vi "VIH HelpGen - Build - Project File Paths Container.vi"(6 "cmd (get)":enum16{"get", "set"}(ring), 9 "HTML Paths in":path[](array[path]), 11 "Item Paths in":path[](array[path])) -> (1 "HTML Paths":path[](array[path]), 2 "Item File Names":string[](array[string]), 3 "Item Paths":path[](array[path]))   [LabVIEW 2014]
doc: "::: VI Helpeks :::\nCopyright (c) 2000-2026 Konstantin Shifershteyn. All rights reserved."
panel:
  # "VI Helpeks\nCopyright (c) 2012-2026 Konstantin Shifershteyn"
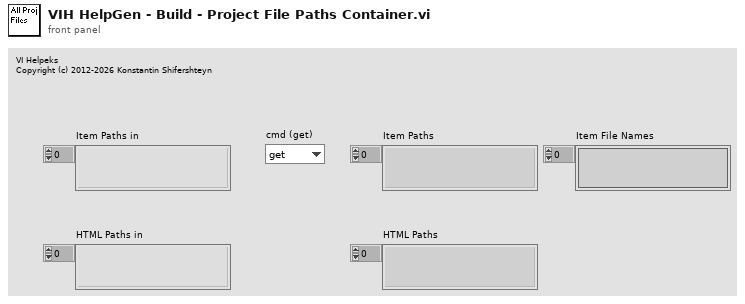
[diagram p1: front panel]
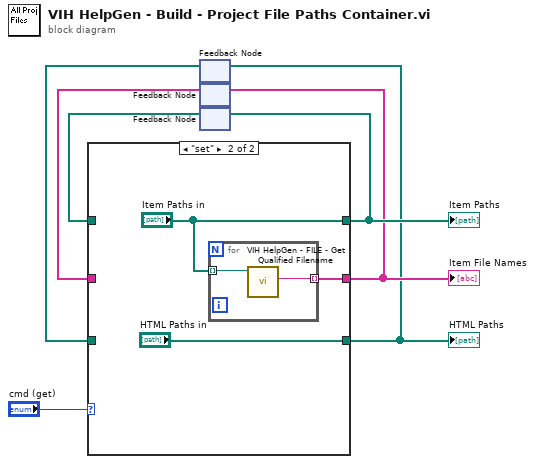
[diagram p0: block diagram]
diagram:
  n1 = feedback #1() -> (w1:path[])  [unwired: 1 in]
  n2 = feedback #2() -> (w3:string[])  [unwired: 1 in]
  n3 = feedback #3() -> (w5:path[])  [unwired: 1 in]
  n4 = case shown="\"set\"" "cmd (get)" {
    tunnel: [w10 "Item Paths in"] -> w6
    tunnel: [w9 w12] -> w4
    tunnel: [w8 "HTML Paths in"] -> w2
    tunnel: w5 -> [w10 _]
    tunnel: w3 -> [w9 _]
    tunnel: w1 -> [w8 _]
    frame "get" {
    }
    frame "set" {
      n5 = for {
        tunnel: "Item Paths in" -> [w15] mode=indexing
        tunnel: [w14] -> w12 mode=indexing
        n6 = call "VIH HelpGen - FILE - Get Qualified Filename.vi"("File Path"=w15) -> ("Qualified name"=w14:string)  [unwired: 9 in, 1 out]
      }
    }
  }
  "Item Paths" <- w6
  "HTML Paths" <- w2
  "Item File Names" <- w4
  n7 = feedback-in #1(w2) -> ()
  n8 = feedback-in #2(w4) -> ()
  n9 = feedback-in #3(w6) -> ()
